vi "Set Cursor.vi"(8 "error in (no error)":errorcluster, 10 "UI Refs":T1, 11 "Visible(F)":bool) -> (0 "error out":errorcluster)   [LabVIEW 2025, in "XY Plotter.lvlib" / "XY Plotter.lvclass"]
uses:
  XY Plotter.lvclass
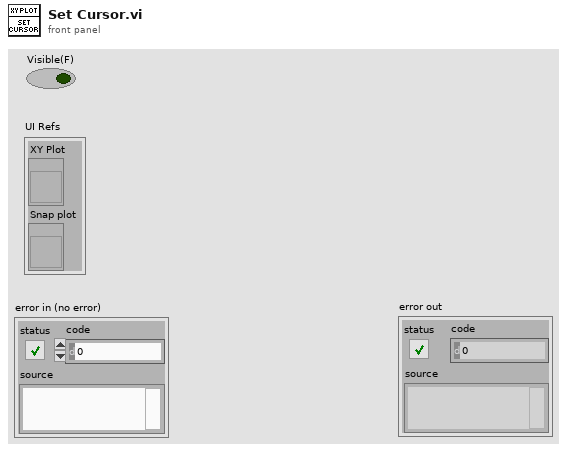
[diagram p1: front panel]
types:
  T1 = cluster{"XY Plot":refnum<vi>, "Snap plot":refnum<vi>}
  T2 = cluster{"Name":string, "Color":u32, "Style":u8, "Point Style":u8, "Name Visible":bool, "Allow Drag":bool, "Cursor Mode":u32, "Plot":i32, "Index":i32, "Position":cluster{"X":dbl, "Y":dbl}, "X Scale":u32, "Y Scale":u32, "Watch Plots":i32[], "Watch All Plots":bool, "Plot Area":i32, "Label Offset":cluster{"X":dbl, "Y":dbl}}
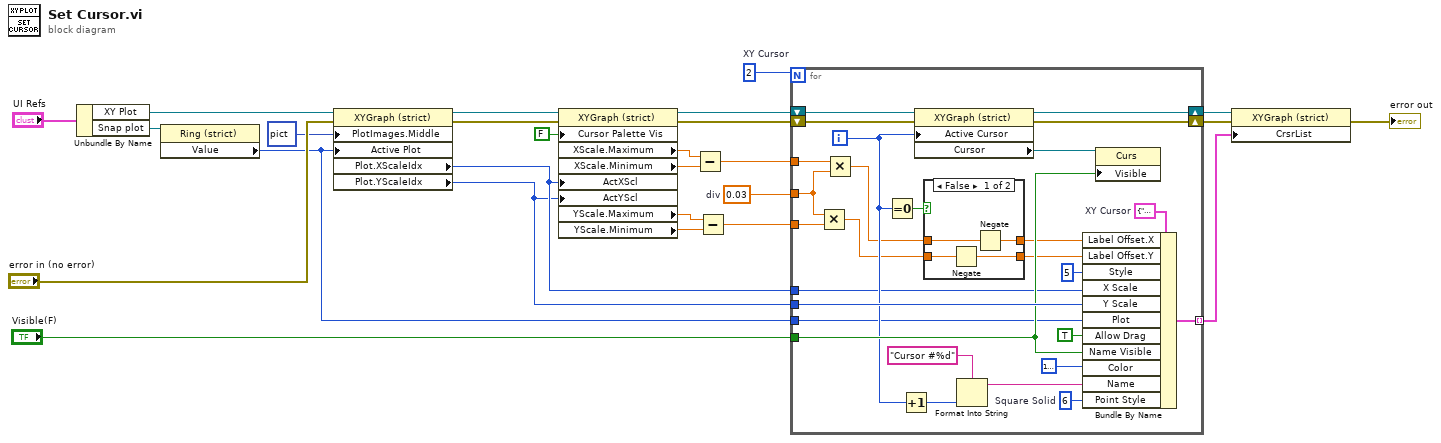
[diagram p0: block diagram]
diagram:
  w6 = 0.03  # div
  w23 = 2  # XY Cursor
  n1 = Unbundle By Name("UI Refs") -> ("XY Plot"=w2:refnum<vi>, "Snap plot"=w1:refnum<vi>)
  n2 = property class="Ring (strict)"(reference=w1) -> ("Value"=w8:u16)  [unwired: 1 in, 2 out]
  n3 = property class="XYGraph (strict)"(reference=w2, error in="error in (no error)", "PlotImages.Middle"=picture data[5B] ("Plot Images:Middle"), "Active Plot"=w8) -> (reference out=w22:refnum<vi>, error out=w17:errorcluster, "Plot.XScaleIdx"=w21:u32, "Plot.YScaleIdx"=w20:u32)
  n4 = property class="XYGraph (strict)"(reference=w22, error in=w17, "Cursor Palette Vis"=FALSE ("Cursor Legend Visible"), "ActXScl"=w21, "ActYScl"=w20) -> (reference out=w13:refnum<vi>, error out=w11:errorcluster, "XScale.Maximum"=w19:dbl, "XScale.Minimum"=w26:dbl, "YScale.Maximum"=w24:dbl, "YScale.Minimum"=w25:dbl)
  n5 = Subtract(x=w19, y=w26) -> (x-y=w9:dbl)
  n6 = Subtract(x=w24, y=w25) -> (x-y=w7:dbl)
  n7 = for {
    N: w23 -> [_]
    tunnel: [w53] -> w14 mode=indexing
    tunnel: w9 -> [w32]
    tunnel: w21 -> [w35]
    tunnel: w20 -> [w44]
    tunnel: "Visible(F)" -> [w40]
    tunnel: w8 -> [w28]
    shift-right: [w46] -> w12
    shift-left: w13 -> [w49]
    shift-right: [w45] -> w10
    shift-left: w11 -> [w48]
    tunnel: w7 -> [w29]
    tunnel: w6 -> [w30]
    i -> [w39]
    w27 = u8 6  # Square Solid
    w50 = T2 {"Name"="", "Color"=0, "Style"=0, "Point Style"=0, "Name Visible"=FALSE, "Allow Drag"=FALSE, "Cursor Mode"=0, "Plot"=0, "Index"=0, "Position"={"X"=0.0, "Y"=0.0}, "X Scale"=0, "Y Scale"=0, "Watch Plots"=[], "Watch All Plots"=FALSE, "Plot Area"=0, "Label Offset"={"X"=0.0, "Y"=0.0}}  # XY Cursor
    n8 = Multiply(x=w30, y=w29) -> (x*y=w33:dbl)
    n9 = Multiply(x=w32, y=w30) -> (x*y=w31:dbl)
    n10 = Equal To 0?(x=w39) -> (x = 0?=w38:bool)
    n11 = Increment(x=w39) -> (x+1=w51:i32)
    n12 = property class="XYGraph (strict)"(reference=w49, error in=w48, "Active Cursor"=w39) -> (reference out=w46:refnum<vi>, error out=w45:errorcluster, "Cursor"=w47:refnum<vi>)
    n13 = case shown="False" w38 {
      tunnel: w31 -> [w55 w59]
      tunnel: w33 -> [w57 w58]
      tunnel: [w54 w59] -> w36
      tunnel: [w56 w58] -> w37
      frame False {
        n14 = Negate(x=w57) -> (-x=w56:dbl)
        n15 = Negate(x=w55) -> (-x=w54:dbl)
      }
      frame True {
      }
    }
    n16 = Format Into String(format string="Cursor #%d", w51) -> (resulting string=w42:string)  [unwired: 2 in, 1 out]
    n17 = Bundle By Name(cluster=w50, "Label Offset.X"=w36, "Label Offset.Y"=w37, "Style"=u8 5, "X Scale"=w35, "Y Scale"=w44, "Plot"=w28, "Allow Drag"=TRUE, "Name Visible"=w40, "Color"=u32 16777228 ("Plot.Plot Color"), "Name"=w42, "Point Style"=w27) -> (w53:T2)
    n18 = property class="Curs"(reference=w47, "Visible"=w40) -> ()  [unwired: 1 in, 2 out]
  }
  n19 = property class="XYGraph (strict)"(reference=w12, error in=w10, "CrsrList"=w14) -> (error out=→"error out":errorcluster)  [unwired: 1 out]
